vi "Main.vi"() -> ()   [LabVIEW 2026]
uses:
  <vilib>/Analysis/baseanly.llb/Mean (DBL).vi
  temperature global.vi
  IVCentral Heater Global.vi
  <vilib>/Analysis/NI_AALBase.lvlib
panel:
  out "Date &Time":string
  in  "Report":bool
  out "Temperatures":dbl[](array[numeric])
  out "TC LOWER":dbl
  out "TC UPPER":dbl
  in  "Thermal Conductivity Settings":T1
  out "Average Thermal conductivity":dbl
  in  "Update Period(S)":u32=2
  in  "Test ID/Name":string
  in  "Set Plate Tempearture(C)":T2
  in  "Log In Button":bool
  out "Current(Central Heater)":dbl
  out "Voltage(Central Heater)":dbl format="%#_3g"
  out "Login Status":string
  in  "stop":bool
  in  "Tab Control":enum32{"Main"}(tab)
  out "Lower Cold Plate":cluster{"LC T1":dbl, "LC T2":dbl, "LC T3":dbl}
  out "Lower Cooling ON":bool
  out "Upper Cooling ON":bool
  out "Heating ON":bool
  in  "Delete Values":bool
  out "XY Graph":cluster{"DATA":dbl[], "DATA":dbl[]}[](graph)
  in  "Graph Type":u16(ring) items=["Thermalconductivity", "Temperature"]
  out "Upper Cold Plate":cluster{"UC T1":dbl, "UC T2":dbl, "UC T3":dbl}
  out "Upper Hot Plate":cluster{"UH T1":dbl, "UH T2":dbl, "UH T3":dbl}
  out "Lower Hot Plate":cluster{"LH T1":dbl, "LH T2":dbl, "LH T3":dbl}
  # "THERMALCONDUCTIVITY  TEST SYSTEM"
  # "Status"
  # "Lower Cold Plate Temperature"
  # "Upper Cold Plate Temperature"
  # "Hot Plate Temperature"
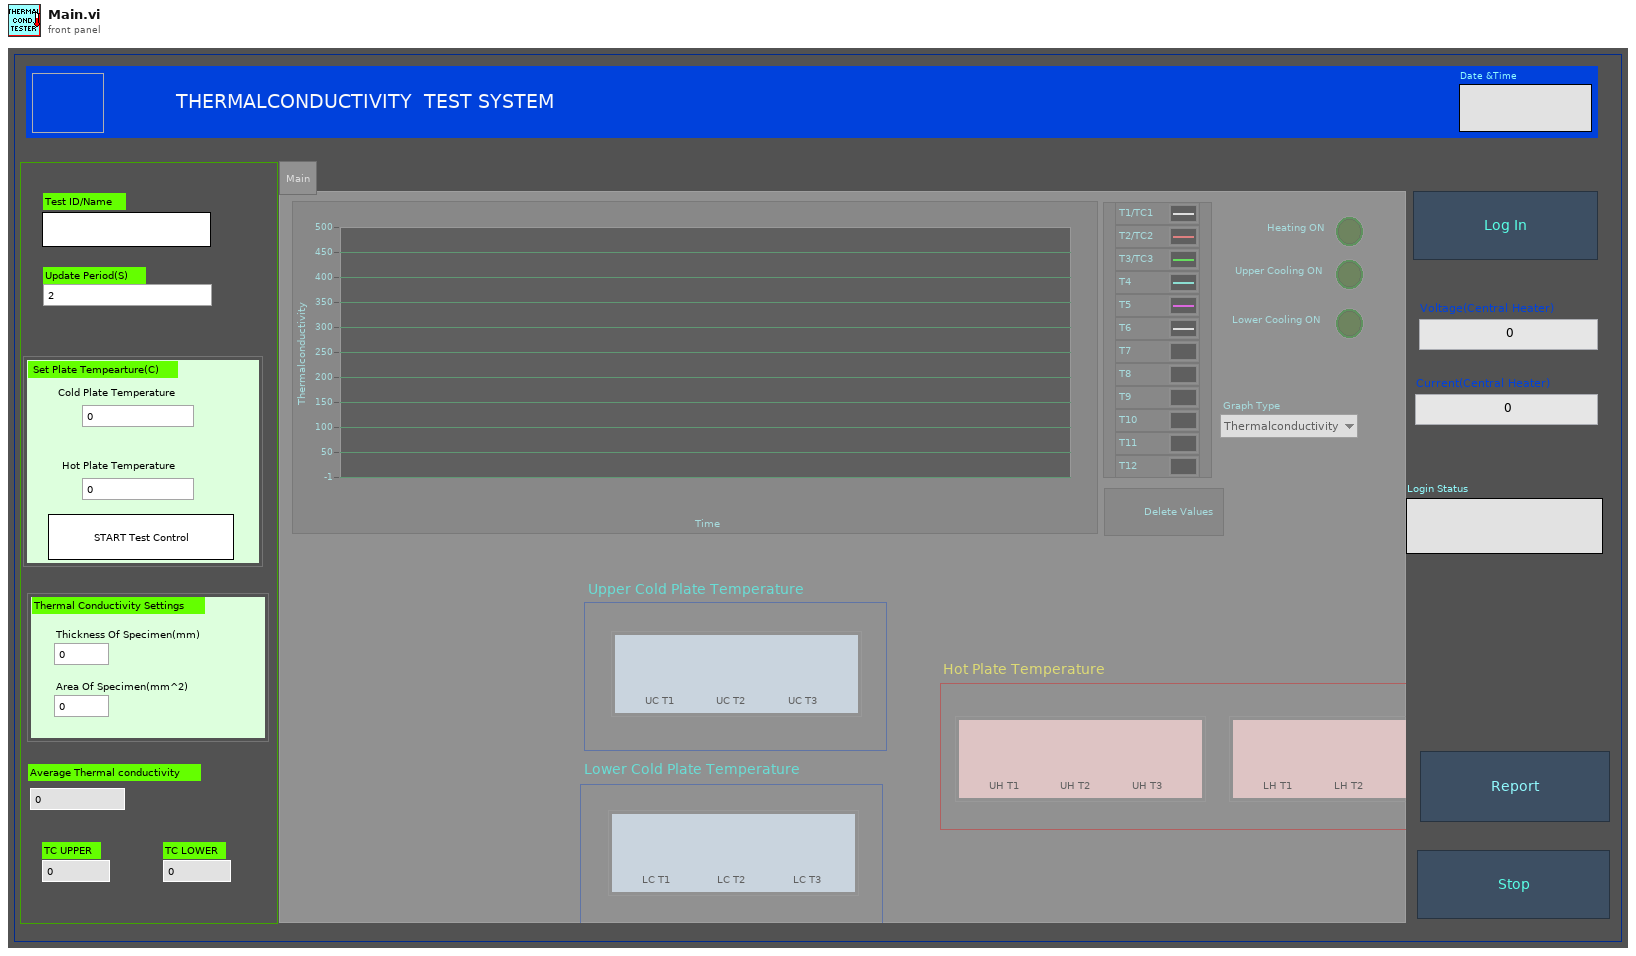
[diagram p1: front panel]
types:
  T1 = cluster{"Thickness Of Specimen(mm)":dbl, "Area Of Specimen(mm^2) ":dbl}
  T2 = cluster{"Cold Plate Temperature":dbl, "Hot Plate Temperature":dbl, "Set Temp":bool}
  T3 = enum8{"Enabled", "Disabled", "Disabled and Grayed Out"}
  T4 = cluster{"Temperatures":dbl, "Temperatures":dbl, "Temperatures":dbl}
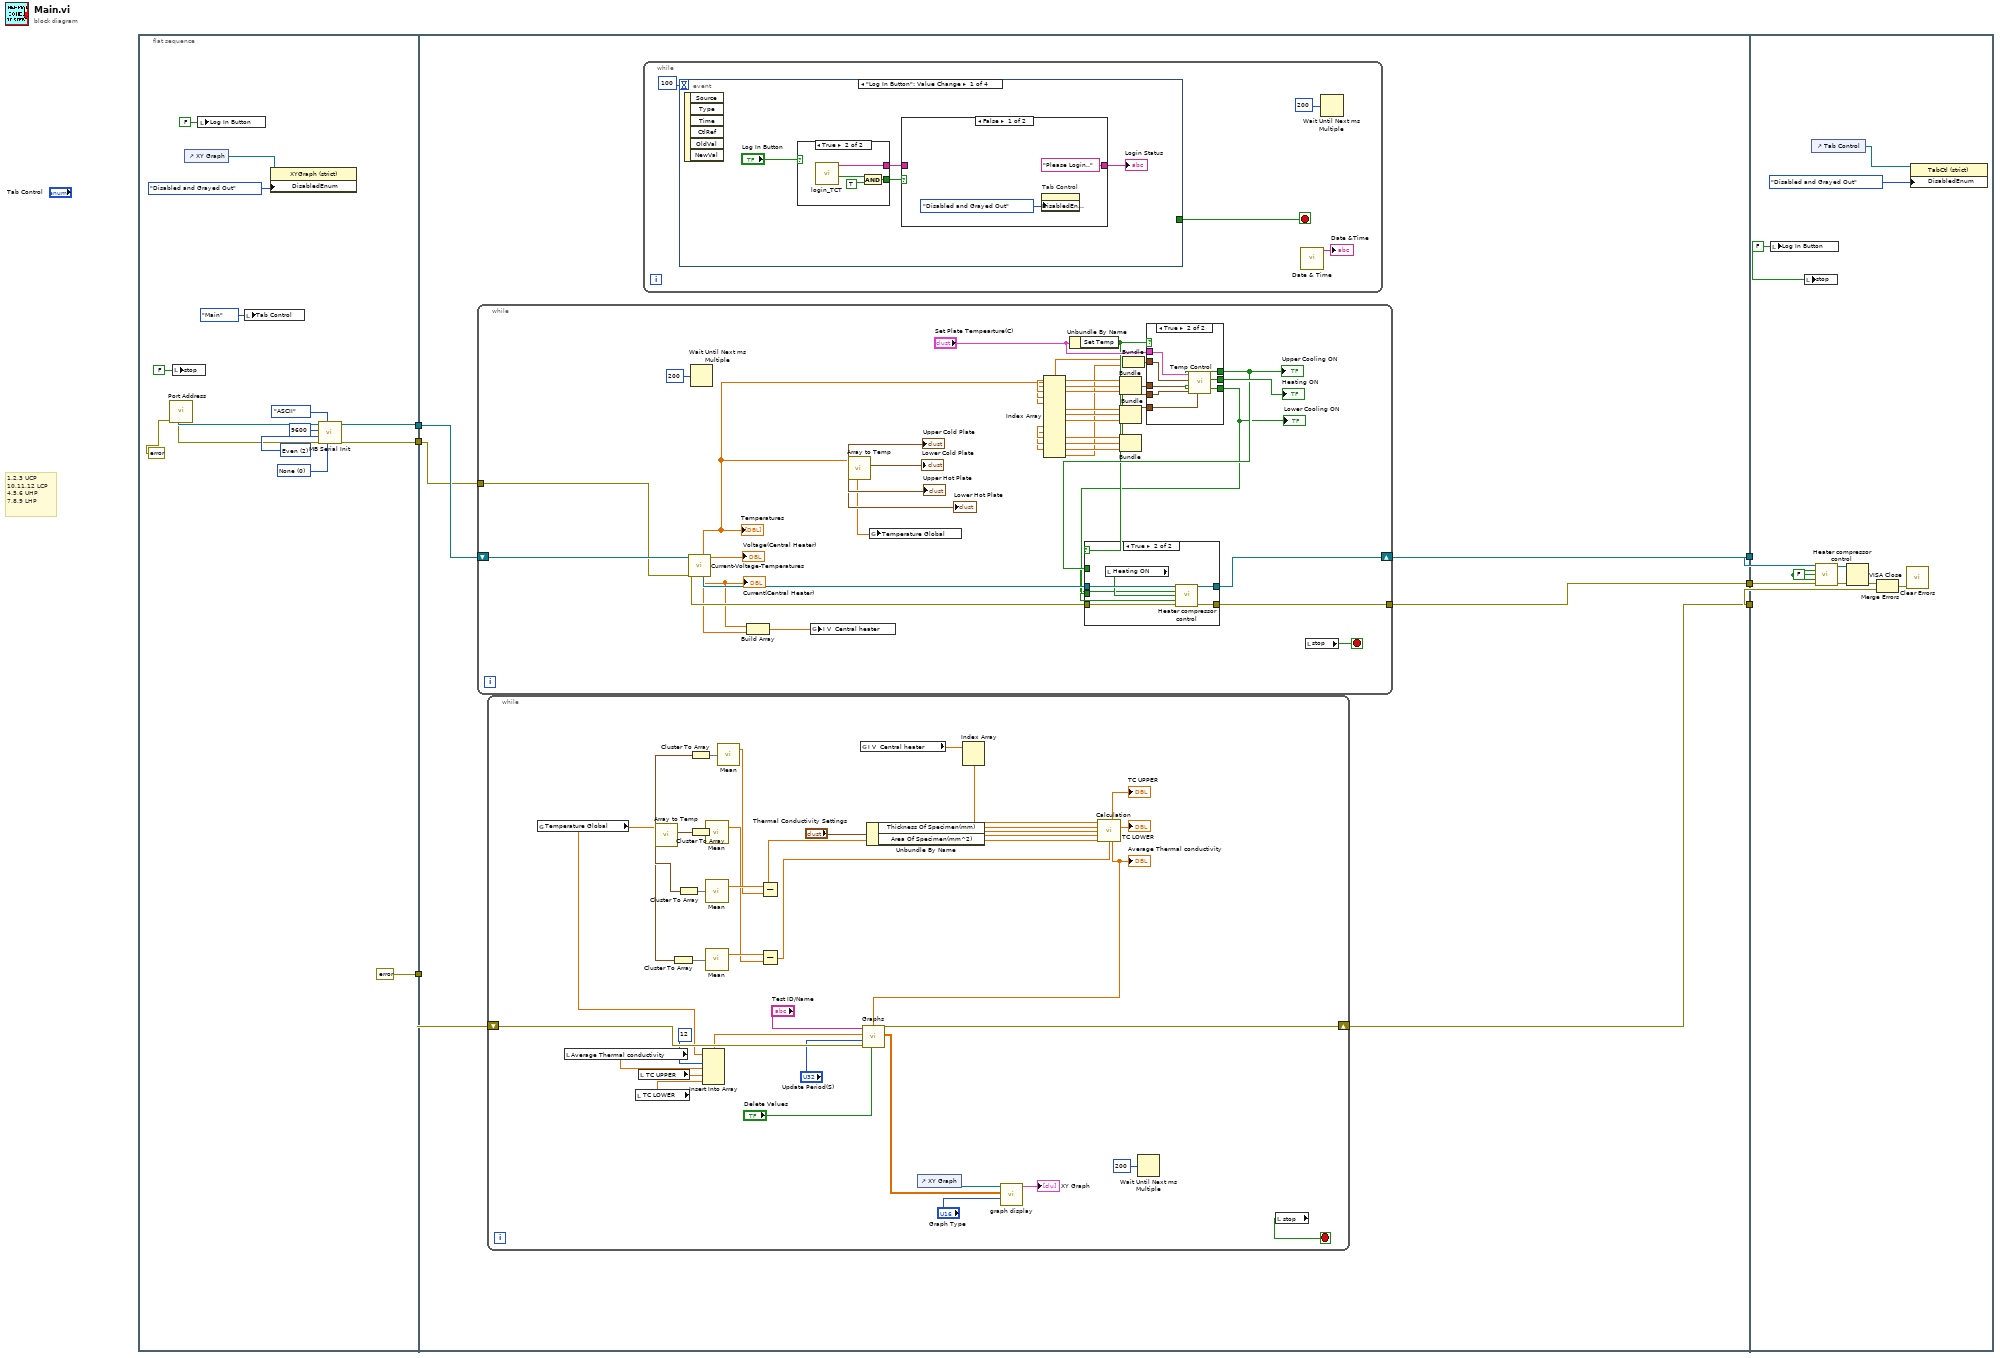
[diagram p0: block diagram]
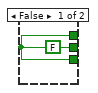
[diagram p2: hidden frame]
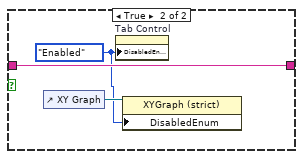
[diagram p5: hidden frame]
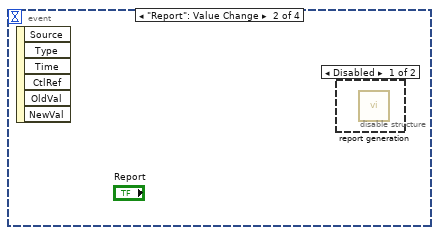
[diagram p6: hidden frame]
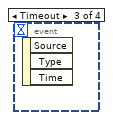
[diagram p8: hidden frame]
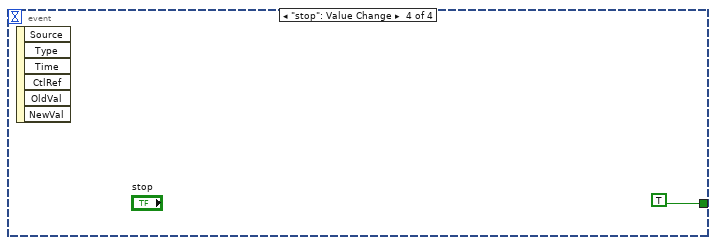
[diagram p9: hidden frame]
diagram:
  # "1,2,3 UCP\n10,11,12 LCP\n4,5,6 UHP\n7,8,9 LHP"
  n1 = flat-sequence {
    tunnel: [w19] -> w6
    tunnel: [w18] -> w5
    tunnel: [errorcluster {"status"=FALSE, "code"=0, "source"=""} ("error constant")] -> w4
    tunnel: w6 -> [w27]
    tunnel: w5 -> [w26]
    tunnel: w4 -> [w25]
    tunnel: [w24] -> w3
    tunnel: [w23] -> w2
    tunnel: [w22] -> w1
    tunnel: w3 -> [w147]
    tunnel: w2 -> [w148]
    tunnel: w1 -> [w143]
    frame #0 {
      w13 = u16 0 items=["None", "XON/XOFF", "RTS/CTS", "XON/XOFF & RTS/CTS", "DTR/DSR", "XON/XOFF & DTR/DSR"] ("Flow Control")
      w14 = u16 2 items=["None", "Odd", "Even", "Mark", "Space"] ("Parity")
      n2 = call "Port Address.vi"("error in"=errorcluster {"status"=FALSE, "code"=0, "source"=""} ("error constant")) -> ("error out"=w10:errorcluster, "Visa Resource"=w12:refnum<visa-resource-name>)  [unwired: 8 in, 1 out]
      n3 = local write "stop"(FALSE) -> ()
      n4 = control-ref of="XY Graph"() -> (w9:refnum<vi>)
      n5 = local write "Log In Button"(FALSE ("Log In Button")) -> ()
      n6 = local write "Tab Control"(enum32{"Main"}."Main" ("Tab Control")) -> ()
      n7 = property class="XYGraph (strict)"(reference=w9, "DisabledEnum"=T3."Disabled and Grayed Out" ("Disabled")) -> ()  [unwired: 1 in, 2 out]
      n8 = call <userlib>:"MB Serial Init.vi"("Flow Control"=w13, "Mode"=enum16{"RTU", "ASCII"}."ASCII", "error in (no error)"=w10, "Parity"=w14, "Baud Rate"=u32 9600, "VISA resource name"=w12) -> ("error out"=w18:errorcluster, "VISA resource name out"=w19:refnum<visa-resource-name>)  [unwired: 4 in]
    }
    frame #1 {
      n9 = while {
        shift-right: [w97] -> w24
        shift-left: w27 -> [w102]
        tunnel: w26 -> [w101]
        tunnel: [w99] -> w22
        stop <- w103 stop-if-true
        n10 = call "Current-Voltage-Temperatures.vi"("VISA resource name"=w102, "error in"=w101) -> ("VISA resource name out"=w98:refnum<visa-resource-name>, "Temperatures"=w73:dbl[], "voltage output"=w68:dbl, "CURRENT mA"=w69:dbl, "error out"=w100:errorcluster)  [unwired: 9 in]
        "Voltage(Central Heater)" <- w68
        "Current(Central Heater)" <- w69
        "Temperatures" <- w73
        n11 = Wait Until Next ms Multiple(millisecond multiple=u32 200 ("millisecond timer value")) -> ()  [unwired: 1 out]
        n12 = Build Array(w69, w68) -> (w70:dbl[])
        n13 = global write "IVCentral Heater Global.vi" "I V  Central heater"(w70) -> ()
        n14 = call "Array to Temp.vi"("Temperatures"=w73) -> ("LHP"=→"Lower Hot Plate":cluster{"LH T1":dbl, "LH T2":dbl, "LH T3":dbl}, "UHP"=→"Upper Hot Plate":cluster{"UH T1":dbl, "UH T2":dbl, "UH T3":dbl}, "LCP"=→"Lower Cold Plate":cluster{"LC T1":dbl, "LC T2":dbl, "LC T3":dbl}, "UCP"=→"Upper Cold Plate":cluster{"UC T1":dbl, "UC T2":dbl, "UC T3":dbl}, "Temperatures"=w72:dbl[])  [unwired: 4 in]
        n15 = global write "temperature global.vi" "Temperature Global"(w72) -> ()
        n16 = Index Array(array=w73) -> (element #1=w92:dbl, element #2=w91:dbl, element #3=w90:dbl, element #4=w89:dbl, element #5=w88:dbl, element #6=w87:dbl, element #7=w86:dbl, element #8=w85:dbl, element #9=w84:dbl, element #10=w83:dbl, element #11=w82:dbl)  [unwired: 12 in, 1 out]
        n17 = Unbundle By Name("Set Plate Tempearture(C)") -> ("Set Temp"=w93:bool)
        n18 = Bundle("Temperatures"=w92, "Temperatures"=w91, "Temperatures"=w90) -> (w79:T4)  [unwired: 1 in]
        n19 = Bundle("Temperatures"=w89, "Temperatures"=w88, "Temperatures"=w87) -> (w78:T4)  [unwired: 1 in]
        n20 = Bundle("Temperatures"=w86, "Temperatures"=w85, "Temperatures"=w84) -> (w80:T4)  [unwired: 1 in]
        n21 = Bundle("Temperatures"=w83, "Temperatures"=w82) -> (w81:cluster{"Temperatures":dbl, "Temperatures":dbl})  [unwired: 1 in]
        n22 = case shown="True" w93 {
          tunnel: "Set Plate Tempearture(C)" -> [_ w113]
          tunnel: [w105 w112] -> w96
          tunnel: [w105 w111] -> w94
          tunnel: [w105 w110] -> w71
          tunnel: w81 -> [_ w109]
          tunnel: w80 -> [_ w108]
          tunnel: w79 -> [_ w107]
          tunnel: w78 -> [_ w106]
          frame False {
            w105 = FALSE
          }
          frame True {
            n23 = call "Temp Control.vi"("Lower Hot Plate"=w108, "Upper Hot Plate"=w106, "Upper Cold Plate"=w107, "Lower Cold Plate"=w109, "Plates Temp Setting"=w113) -> ("LCP Compr On"=w110:bool, "UHP Heater On"=w112:bool, "UCP Compr On"=w111:bool)  [unwired: 4 in]
          }
        }
        "Heating ON" <- w96
        "Upper Cooling ON" <- w94
        "Lower Cooling ON" <- w71
        n24 = case shown="True" w93 {
          tunnel: w100 -> [w114 w122]
          tunnel: [w114 w121] -> w99
          tunnel: w98 -> [w115 w120]
          tunnel: [w115 w119] -> w97
          tunnel: w94 -> [_ w117]
          tunnel: w71 -> [_ w116]
          frame False {
          }
          frame True {
            n25 = local read "Heating ON"() -> (w118:bool)
            n26 = call "Heater compressor control.vi"("VISA resource name"=w120, "UCP"=w117, "Heater on"=w118, "LCP"=w116, "error in"=w122) -> ("VISA resource name out"=w119:refnum<visa-resource-name>, "error out"=w121:errorcluster)  [unwired: 9 in]
          }
        }
        n27 = local read "stop"() -> (w103:bool)
      }
      n28 = while {
        shift-right: [w67] -> w23
        shift-left: w25 -> [w66]
        stop <- w65 stop-if-true
        n29 = global read "temperature global.vi" "Temperature Global"() -> (w32:dbl[])
        n30 = local read "Average Thermal conductivity"() -> (w54:dbl)
        n31 = local read "TC LOWER"() -> (w36:dbl)
        n32 = local read "TC UPPER"() -> (w37:dbl)
        n33 = call "Array to Temp.vi"("Temperatures"=w32) -> ("LHP"=w42:cluster{"LH T1":dbl, "LH T2":dbl, "LH T3":dbl}, "UHP"=w44:cluster{"UH T1":dbl, "UH T2":dbl, "UH T3":dbl}, "LCP"=w41:cluster{"LC T1":dbl, "LC T2":dbl, "LC T3":dbl}, "UCP"=w43:cluster{"UC T1":dbl, "UC T2":dbl, "UC T3":dbl})  [unwired: 4 in, 1 out]
        n34 = Cluster To Array(cluster=w42) -> (array=w48:dbl[])
        n35 = Cluster To Array(cluster=w44) -> (array=w53:dbl[])
        n36 = Cluster To Array(cluster=w43) -> (array=w52:dbl[])
        n37 = Cluster To Array(cluster=w41) -> (array=w47:dbl[])
        n38 = Insert Into Array "Insert Into Array"(array=w32, index=12, new element #1=w54, new element #2=w37, new element #3=w36) -> (w55:dbl[])
        n39 = call-poly <vilib>:"Mean.vi"("X"=w47) -> ("mean"=w45:dbl)  [unwired: 1 out]
        n40 = call-poly <vilib>:"Mean.vi"("X"=w53) -> ("mean"=w51:dbl)  [unwired: 1 out]
        n41 = call-poly <vilib>:"Mean.vi"("X"=w48) -> ("mean"=w46:dbl)  [unwired: 1 out]
        n42 = call-poly <vilib>:"Mean.vi"("X"=w52) -> ("mean"=w50:dbl)  [unwired: 1 out]
        n43 = Subtract(x=w51, y=w50) -> (x-y=w49:dbl)
        n44 = Subtract(x=w46, y=w45) -> (x-y=w40:dbl)
        n45 = global read "IVCentral Heater Global.vi" "I V  Central heater"() -> (w29:dbl[])
        n46 = Unbundle By Name("Thermal Conductivity Settings") -> ("Thickness Of Specimen(mm)"=w58:dbl, "Area Of Specimen(mm^2)"=w57:dbl)
        n47 = control-ref of="XY Graph"() -> (w35:refnum<vi>)
        n48 = Index Array(array=w29) -> (element #1=w31:dbl, element #2=w30:dbl)  [unwired: 2 in]
        n49 = call "Calculation.vi"("Current(i)"=w31, "Voltage(v)"=w30, "Thickness Of Specimen(l)"=w58, "Area of specimen(m2)"=w57, "UPPER(Th-Tc)"=w49, "LOWER(Th-Tc)"=w40) -> ("Themal Conductivity UPPER"=→"TC UPPER":dbl, "Themal Conductivity LOWER"=→"TC LOWER":dbl, "Themal Conductivity avg"=w28:dbl)  [unwired: 6 in, 1 out]
        "Average Thermal conductivity" <- w28
        n50 = call "Graphs.vi"("Delete Values"="Delete Values", "Avg Thermal conductivity"=w28, "error in (no error)"=w66, "Time"="Update Period(S)", "Data In"=w55, "Test ID"="Test ID/Name") -> ("error out"=w67:errorcluster, "DATA"=w63:dbl[][])  [unwired: 3 in, 1 out]
        n51 = call "graph display.vi"("Graph Type"="Graph Type", "DATA"=w63, "XYGraph in"=w35) -> ("Array"=→"XY Graph":cluster{"DATA":dbl[], "DATA":dbl[]}[])  [unwired: 8 in]
        n52 = Wait Until Next ms Multiple(millisecond multiple=u32 200) -> ()  [unwired: 1 out]
        n53 = local read "stop"() -> (w65:bool)
      }
      n54 = while {
        stop <- w125 stop-if-true
        n55 = event shown="[0] \"Log In Button\": Value Change" {
          selector: _ -> [_ _ _ _]
          dyn-events: _ -> [_ _ _ _]
          timeout: 100 -> [_ _ _ _]
          tunnel: [_ _ _ TRUE] -> w125
          event "Log In Button": Value Change {
            n56 = event-data() -> ()  [unwired: 1 in, 6 out]
            n57 = case shown="True" "Log In Button" {
              tunnel: [_ w134] -> w129
              tunnel: [_ w131] -> w128
              frame False {
              }
              frame True {
                n58 = call "login_TCT.vi"() -> ("LOGIN"=w133:bool, "Login String"=w134:string)  [unwired: 10 in]
                n59 = And(x=w133, y=TRUE) -> (x .and. y?=w131:bool)
              }
            }
            n60 = case shown="False" w128 {
              tunnel: ["Please Login.." w139] -> w130
              tunnel: w129 -> [_ w139]
              frame False {
                n61 = property on="Tab Control" class="TabCtl (strict)"("DisabledEnum"=T3."Disabled and Grayed Out" ("Disabled")) -> ()  [unwired: 2 in, 2 out]
              }
              frame True {
                w137 = T3."Enabled" ("Disabled")
                n62 = control-ref of="XY Graph"() -> (w138:refnum<vi>)
                n63 = property on="Tab Control" class="TabCtl (strict)"("DisabledEnum"=w137) -> ()  [unwired: 2 in, 2 out]
                n64 = property class="XYGraph (strict)"(reference=w138, "DisabledEnum"=w137) -> ()  [unwired: 1 in, 2 out]
              }
            }
            "Login Status" <- w130
          }
          event "Report": Value Change {
            n65 = event-data() -> ()  [unwired: 1 in, 6 out]
            n66 = disable-structure shown="Disabled" {
              frame Disabled {
                n67 = call "report generation.vi"() -> ()  [unwired: 12 in]
              }
              frame Enabled {
              }
            }
          }
          event Timeout {
            n68 = event-data() -> ()  [unwired: 1 in, 3 out]
          }
          event "stop": Value Change {
            n69 = event-data() -> ()  [unwired: 1 in, 6 out]
          }
        }
        n70 = call "Date & Time.vi"() -> ("String"=→"Date &Time":string)  [unwired: 11 in]
        n71 = Wait Until Next ms Multiple(millisecond multiple=u32 200 ("millisecond timer value")) -> ()  [unwired: 1 out]
      }
    }
    frame #2 {
      w144 = FALSE
      w151 = FALSE ("Log In Button")
      n72 = local write "Log In Button"(w151) -> ()
      n73 = local write "stop"(w151) -> ()
      n74 = control-ref of="Tab Control"() -> (w141:refnum<vi>)
      n75 = call "Heater compressor control.vi"("VISA resource name"=w147, "UCP"=w144, "Heater on"=w144, "LCP"=w144, "error in"=w143) -> ("VISA resource name out"=w145:refnum<visa-resource-name>, "error out"=w146:errorcluster)  [unwired: 9 in]
      n76 = VISA Close(VISA resource name=w145, error in (no error)=w146) -> (error out=w150:errorcluster)
      n77 = Merge Errors(w150, w148) -> (w149:errorcluster)
      n78 = call <vilib>:"Clear Errors.vi"("error in (no error)"=w149) -> ()  [unwired: 5 in, 2 out]
      n79 = property on="Property Node" class="TabCtl (strict)"(reference=w141, "DisabledEnum"=T3."Disabled and Grayed Out" ("Disabled")) -> ()  [unwired: 1 in, 2 out]
    }
  }
